vi "DNL_Measurement_Spec_DAC.vi"(0 "Start Code":dbl, 1 "Resolution":u16=12, 5 "Stop Code":dbl=4095.0, 7 "Step Size":dbl=1.0, 9 "Settling Time (ms)":u32=10, 11 "Error In":errorcluster, 12 "Reference Voltage":dbl=5.0 format="%#.6p") -> (15 "Error Out":errorcluster)   [LabVIEW 2026, in "Core.lvlib"]
doc: "Configures the measurement parameters required for DAC DNL testing, including code sweep settings, DAC resolution, reference voltage, and settling time."
uses:
  Core.lvlib
  TypeDefs/Enum_Events.ctl
  TypeDefs/Enum_Event_Options.ctl
  TypeDefs/Enum_Notifier_Name.ctl
  TypeDefs/Enum_Notifier_Options.ctl
  TypeDefs/Notification_Clusters/Cluster_DNL_Measurement_Specs.ctl
  TypeDefs/Notification_Clusters/Cluster_INL_Measurement_Specs.ctl
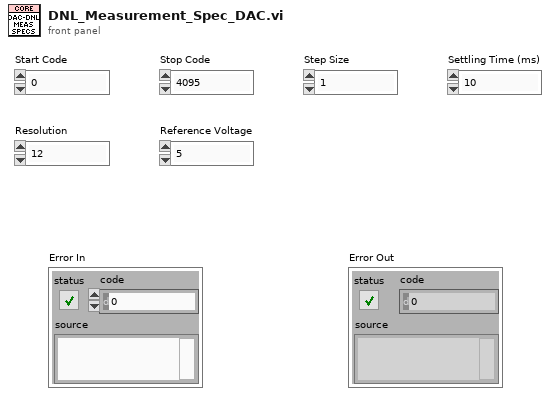
[diagram p1: front panel]
types:
  T1 = typedef "Core.lvlib/Cluster_DNL_Measurement_Specs.ctl" = cluster{" Resolution":u16, "Reference Voltage":dbl, "Settling Time (ms)":u32, "Start":dbl, "Step Size":dbl, "Stop":dbl}
  T2 = typedef "Core.lvlib/Enum_Notifier_Options.ctl" = enum16{"Create", "Send", "Status", "Release"}
  T3 = typedef "Core.lvlib/Enum_Notifier_Name.ctl" = enum16{"Device Type", "Test", "Instrument Spec", "Measurement Spec", "Status"}
  T4 = typedef "Core.lvlib/Enum_Events.ctl" = enum16{"Stop All", "Stop Subpanel", "Stop Test Spec", "Stop Result"}
  T5 = typedef "Core.lvlib/Enum_Event_Options.ctl" = enum16{"Create", "Generate", "Event Ref", "Destroy"}
  T6 = typedef "Core.lvlib/Cluster_INL_Measurement_Specs.ctl" = cluster{" Resolution":u16, "Reference Voltage":dbl, "Settling Time (ms)":u32, "Start":dbl, "Step Size":dbl, "Stop":dbl}
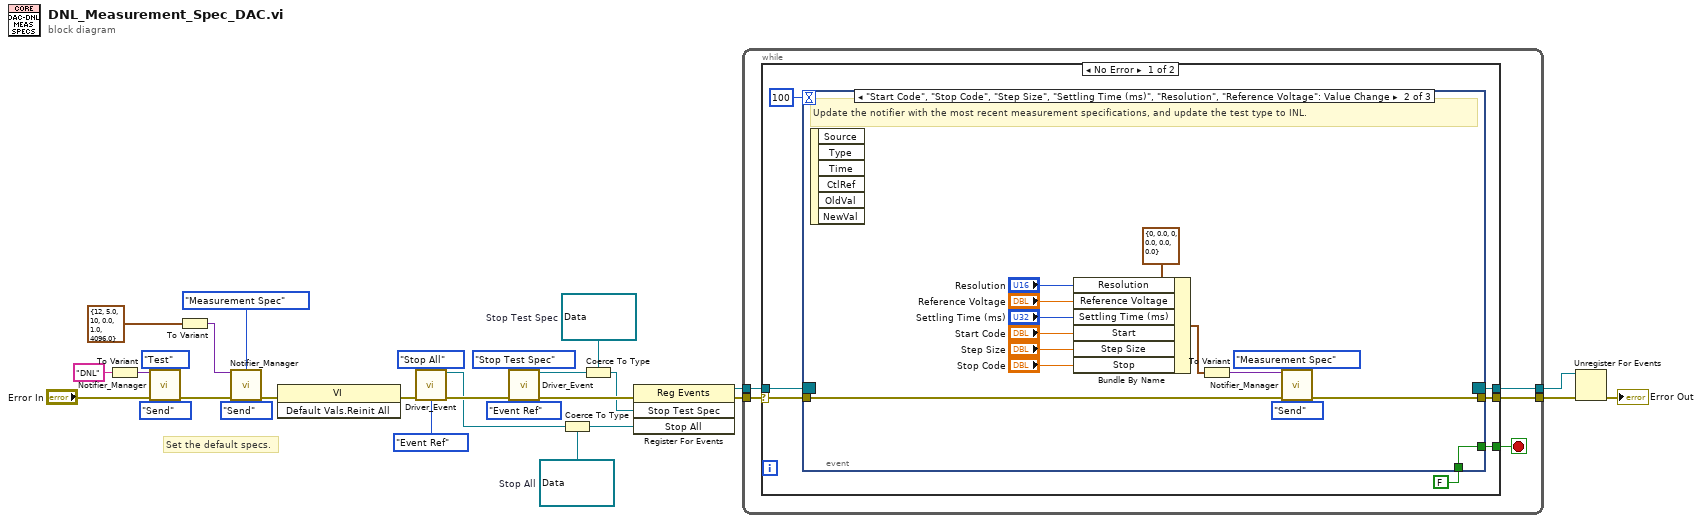
[diagram p0: block diagram]
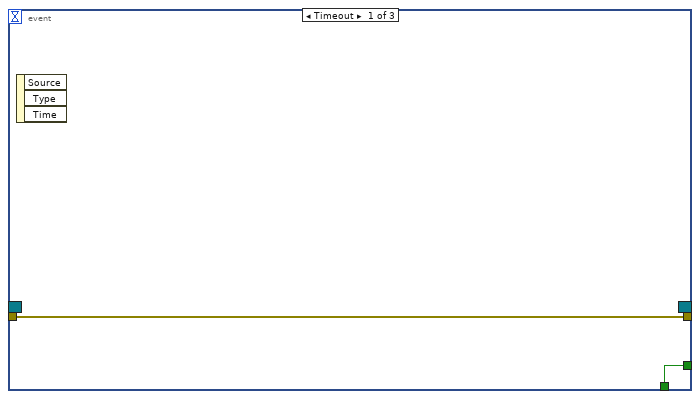
[diagram p2: hidden frame]
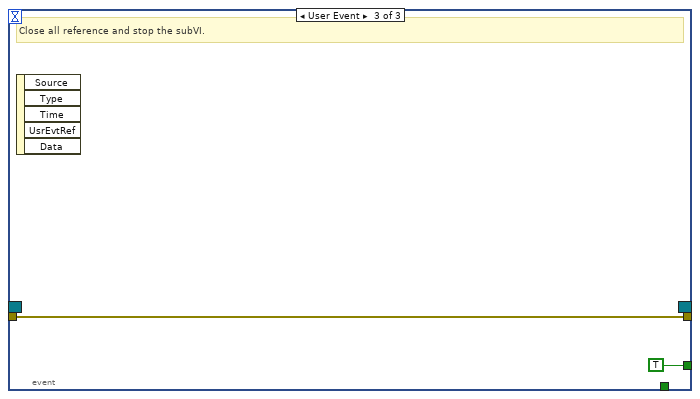
[diagram p3: hidden frame]
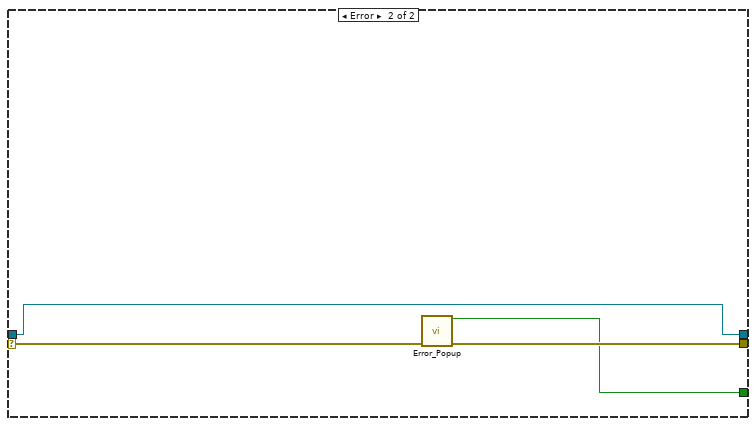
[diagram p4: hidden frame]
diagram:
  w12 = refnum<user-event> refnum  # Stop All
  w21 = refnum<user-event> refnum  # Stop Test Spec
  # "Set the default specs."
  n1 = To Variant(anything="DNL") -> (Variant=w11:variant)
  n2 = call "Notifier_Manager.vi"("Notifier Data"=w11, "Notifier Name"=Enum_Notifier_Name."Test", "Error In"="Error In", "Notifier Options"=Enum_Notifier_Options."Send") -> ("Error Out"=w7:errorcluster)  [unwired: 10 in, 1 out]
  n3 = To Variant(anything=T1 {" Resolution"=12, "Reference Voltage"=5.0, "Settling Time (ms)"=10, "Start"=0.0, "Step Size"=1.0, "Stop"=4096.0} ("Measurement Specs")) -> (Variant=w4:variant)
  n4 = call "Notifier_Manager.vi"("Notifier Data"=w4, "Notifier Name"=Enum_Notifier_Name."Measurement Spec", "Error In"=w7, "Notifier Options"=Enum_Notifier_Options."Send") -> ("Error Out"=w2:errorcluster)  [unwired: 10 in, 1 out]
  n5 = invoke class="VI" method="Default Vals.Reinit All"(error in=w2) -> (error out=w18:errorcluster)  [unwired: 2 in, 2 out]
  n6 = call "Driver_Event.vi"("Event"=Enum_Events."Stop All", "Error In"=w18, "Event Operation"=Enum_Event_Options."Event Ref") -> ("Event Ref"=w14:refnum<user-event>, "Error Out"=w17:errorcluster)  [unwired: 11 in]
  n7 = call "Driver_Event.vi"("Event"=Enum_Events."Stop Test Spec", "Error In"=w17, "Event Operation"=Enum_Event_Options."Event Ref") -> ("Event Ref"=w28:refnum<user-event>, "Error Out"=w27:errorcluster)  [unwired: 11 in]
  n8 = Coerce To Type(0:w14, 1:w12) -> (2:w13:refnum<user-event>)
  n9 = Coerce To Type(0:w28, 1:w21) -> (2:w22:refnum<user-event>)
  n10 = register-events(error in=w27, w22, w13) -> (reference out=w25:refnum<event-registration>, error out=w26:errorcluster)  [unwired: 1 in]
  n11 = while {
    tunnel: w26 -> [w33]
    tunnel: [w34] -> w29
    tunnel: w25 -> [w32]
    tunnel: [w31] -> w23
    stop <- w30 stop-if-true
    n12 = case shown="No Error" w33 {
      selector: w33 -> [w40 w63]
      tunnel: [w41 w62] -> w34
      tunnel: w32 -> [w38 w61]
      tunnel: [w37 w61] -> w31
      tunnel: [w36 w60] -> w30
      frame No Error {
        n13 = event shown="[1] \"Start Code\", \"Stop Code\", \"Step Size\", \"Settling Time (ms)\", \"Resolution\", \"Reference Voltage\": Value Change" {
          selector: w38 -> [_ _ _]
          dyn-events: [_ _ _] -> w37
          timeout: 100 -> [_ _ _]
          tunnel: [w43 w44 w58] -> w41
          tunnel: w40 -> [w43 w56 w58]
          tunnel: [w42 w57 TRUE] -> w36
          tunnel: FALSE -> [w42 w57 _]
          event Timeout {
            n14 = event-data() -> ()  [unwired: 1 in, 3 out]
          }
          event "Start Code", "Stop Code", "Step Size", "Settling Time (ms)", "Resolution", "Reference Voltage": Value Change {
            # "Update the notifier with the most recent measurement specifications, and update the test type to INL."
            n15 = event-data() -> ()  [unwired: 1 in, 6 out]
            n16 = Bundle By Name(cluster=T6 {" Resolution"=0, "Reference Voltage"=0.0, "Settling Time (ms)"=0, "Start"=0.0, "Step Size"=0.0, "Stop"=0.0} ("Measurement Specs"), "Resolution"="Resolution", "Reference Voltage"="Reference Voltage", "Settling Time (ms)"="Settling Time (ms)", "Start"="Start Code", "Step Size"="Step Size", "Stop"="Stop Code") -> (w46:T6)
            n17 = To Variant(anything=w46) -> (Variant=w45:variant)
            n18 = call "Notifier_Manager.vi"("Notifier Data"=w45, "Notifier Name"=Enum_Notifier_Name."Measurement Spec", "Error In"=w56, "Notifier Options"=Enum_Notifier_Options."Send") -> ("Error Out"=w44:errorcluster)  [unwired: 10 in, 1 out]
          }
          event User Event {
            # "Close all reference and stop the subVI."
            n19 = event-data() -> ()  [unwired: 1 in, 5 out]
          }
        }
      }
      frame Error {
        n20 = call "Error_Popup.vi"("Error In"=w63) -> ("Stop?"=w60:bool, "Error Out"=w62:errorcluster)  [unwired: 13 in]
      }
    }
  }
  n21 = Unregister For Events(event registration refnum=w23, error in=w29) -> (error out=→"Error Out":errorcluster)
